vi "Game of Life.vi"() -> ()   [LabVIEW 2021, in "Game of Life.lvlib"]
doc: "InstrumentStudio plug-in example that displays Conway's Game of Life simulation in a graph."
uses:
  Game of Life.lvlib
  <vilib>/Plug-In SDKs/InstrumentStudio/Plugin Events Enum.ctl
  Helpers/Data Cluster.ctl
  Helpers/Configuration.ctl
  Queue Driver/Queue Operations.ctl
  Queue Driver/Queue State and Data.ctl
  User Event Driver/User Event Operations.ctl
  Helpers/Graph Elements.ctl
  <vilib>/Utility/error.llb/DialogType.ctl
  <vilib>/Utility/error.llb/Error Cluster From Error Code.vi
  <vilib>/ErrorRing/Error Ring.xnode
  <vilib>/Plug-In SDKs/InstrumentStudio/Plugin Session.lvclass
  <vilib>/Plug-In SDKs/InstrumentStudio/InstrumentStudio Plugin SDK.lvlib
  Queue Driver/Queue Driver.lvlib
  User Event Driver/User Event Driver.lvlib
panel:
  in  "Tab Control":enum32{"Game Panel", "Events"}(tab)
  in  "width":u32=100 caption="Board width" min=5 max=1000 step=1
  in  "height":u32=100 caption="Board height" min=5 max=1000 step=1
  in  "update interval":u32=500 caption="Update interval (msec)" min=100 max=2000 step=100
  out "generation":u32 caption="Generation"
  out "game of life":T1(graph)
  in  "Start/Stop":bool
  out "Event Record":i32(listbox)=-1
  in  "Session Id":u64
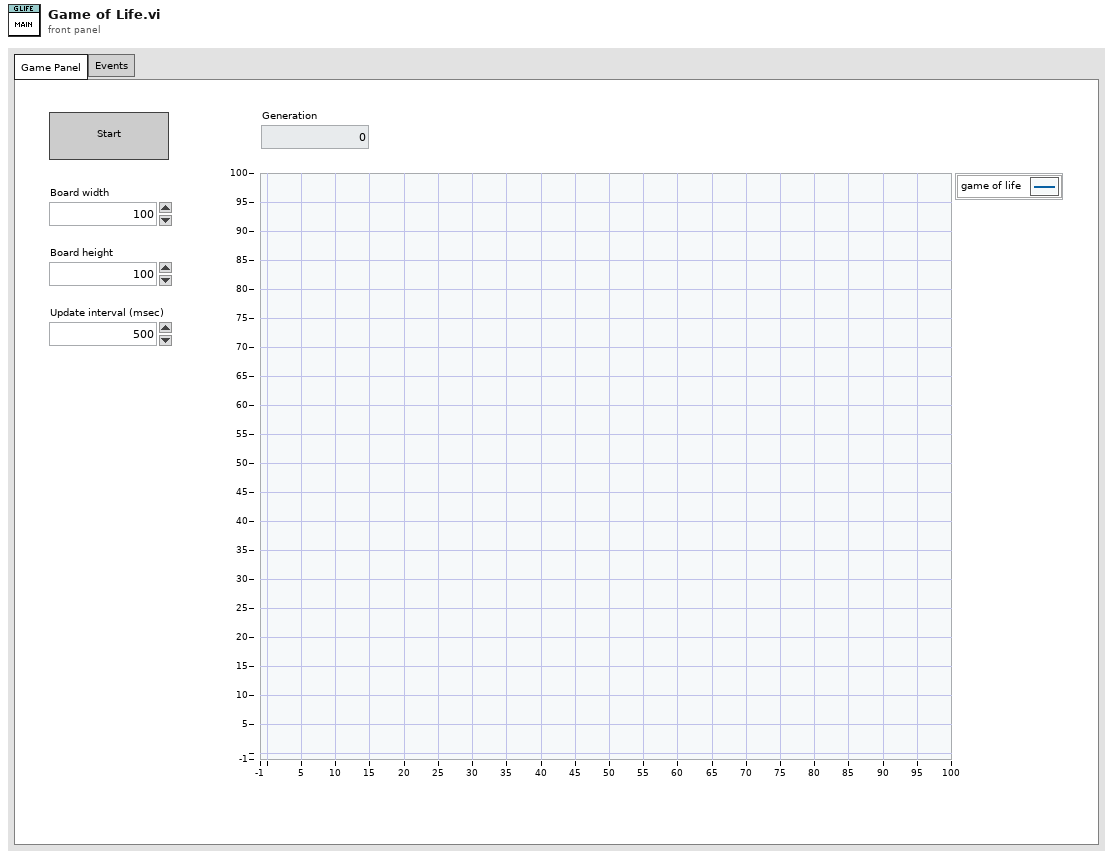
[diagram p1: front panel]
types:
  T1 = typedef "Game of Life.lvlib/Graph Elements.ctl" = cluster{"x data":dbl[], "y data":dbl[]}
  T2 = typedef "Game of Life.lvlib/User Event Driver.lvlib/User Event Operations.ctl" = enum16{"Create", "Destroy", "Get Reference", "Generate"}
  T3 = typedef "Game of Life.lvlib/Queue Driver.lvlib/Queue State and Data.ctl" = cluster{"state":string, "data":variant}
  T4 = typedef "Game of Life.lvlib/Queue Driver.lvlib/Queue Operations.ctl" = enum16{"Create Q", "Enqueue", "Enqueue N", "Enstack", "Enstack N", "Dequeue", "Flush", "Release"}
  T5 = typedef "Game of Life.lvlib/Data Cluster.ctl" = cluster{"configuration":T6, "generation":u32, "cells":bool[][], "event records":string[], "running?":bool, "board update time":timestamp}
  T6 = typedef "Game of Life.lvlib/Configuration.ctl" = cluster{"height":u32, "width":u32, "interval":u32}
  T7 = typedef "InstrumentStudio Plugin SDK.lvlib/Plugin Events Enum.ctl" = enum32{"Shutdown", "Project Saved", "Stop All Outputs", "Generic Message", "Active Pin Map Changed", "Selected Sites Changed"}
  T8 = typedef "InstrumentStudio Plugin SDK.lvlib/Event Registration Refnum.ctl" = refnum<event-registration>
  T9 = cluster{"Event Refnum":T8, "Event Registration Refnum":refnum<event-registration>}
  T10 = enum8{"Enabled", "Disabled", "Disabled and Grayed Out"}
  T11 = typedef "DialogType.ctl" = u16
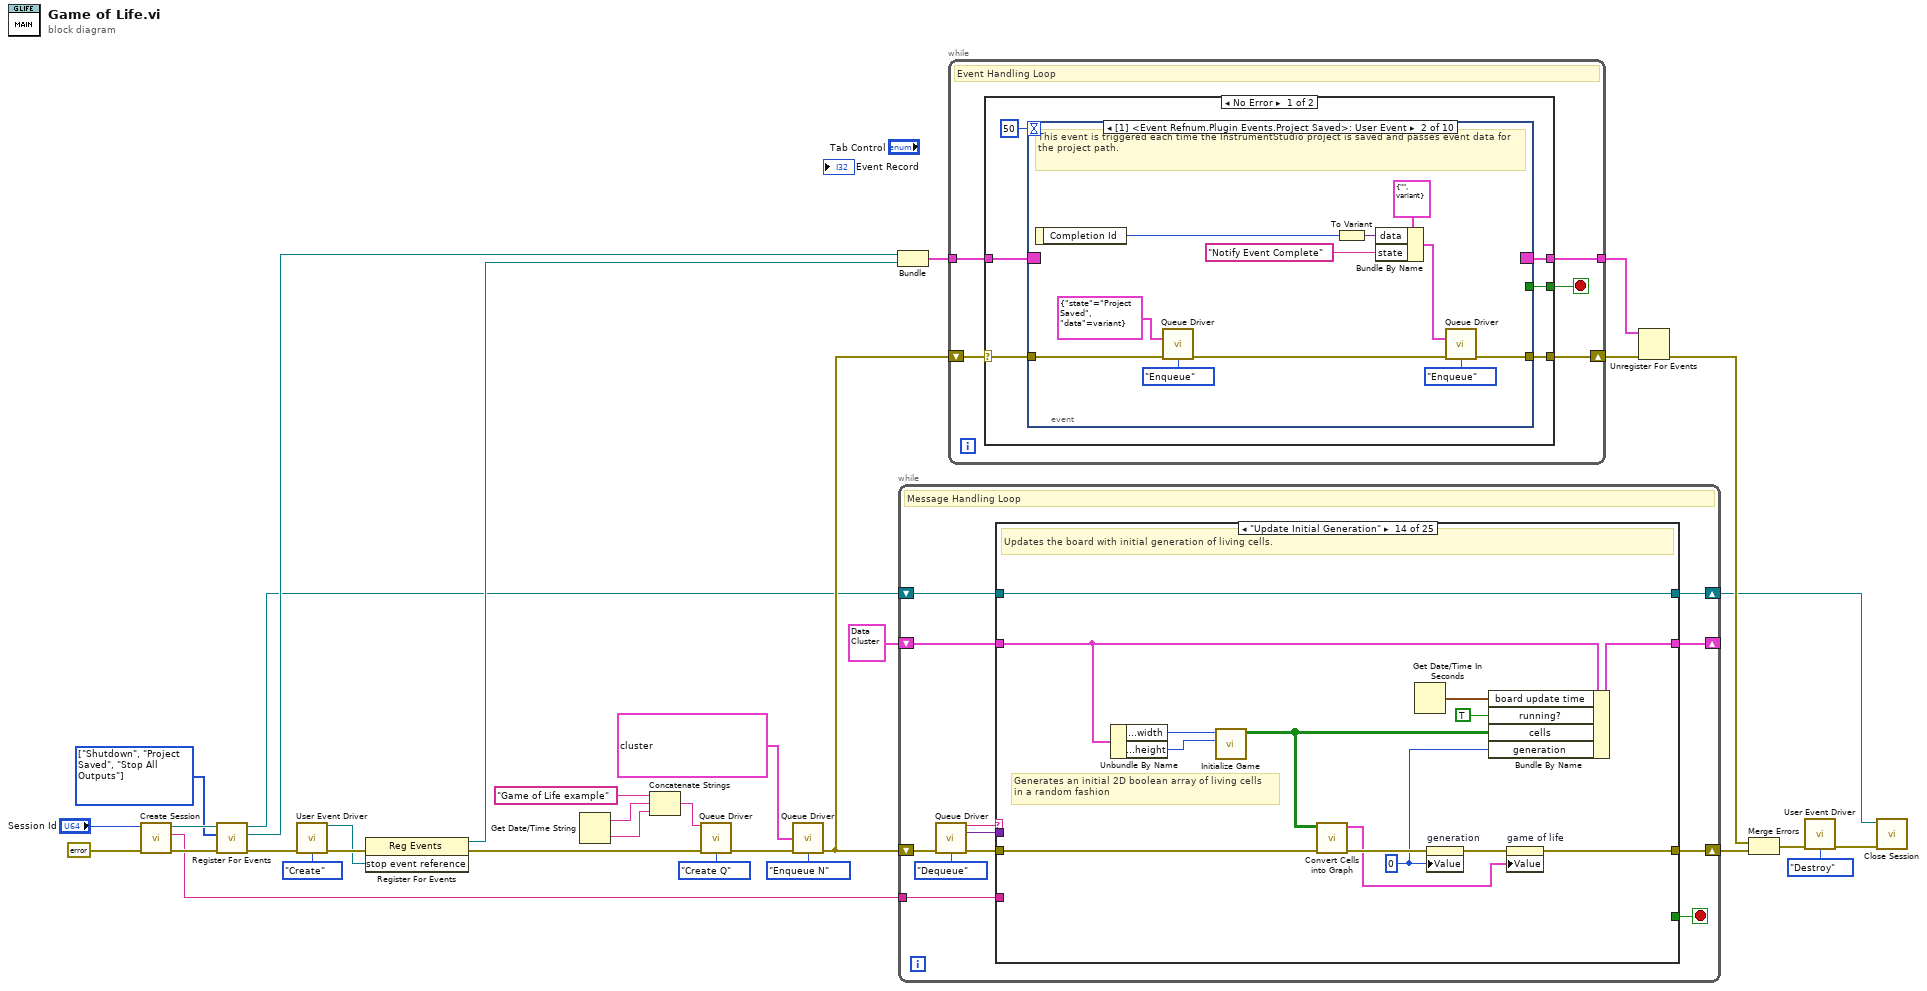
[diagram p0: block diagram]
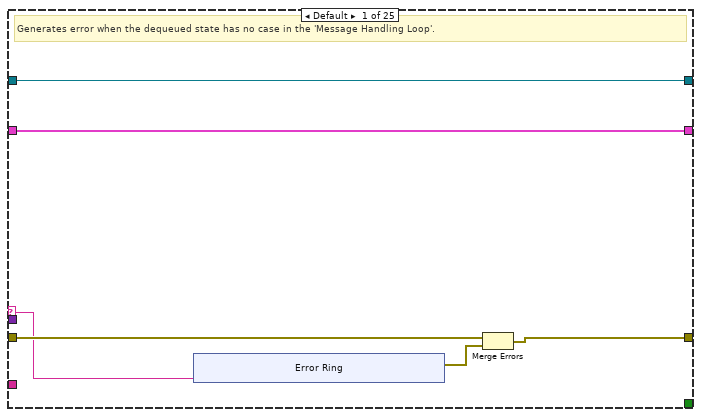
[diagram p2: hidden frame]
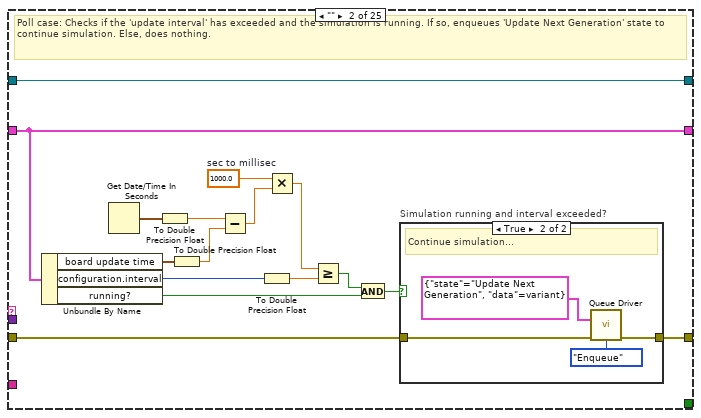
[diagram p3: hidden frame]
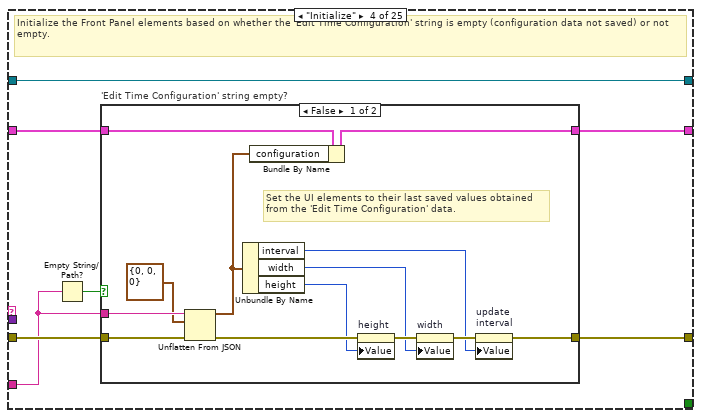
[diagram p6: hidden frame]
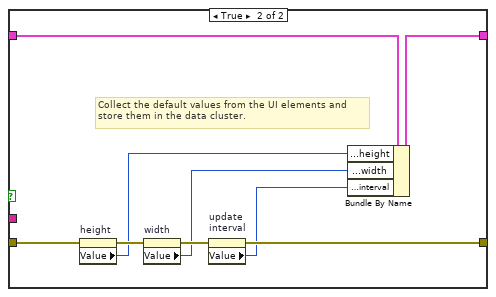
[diagram p7: hidden frame]
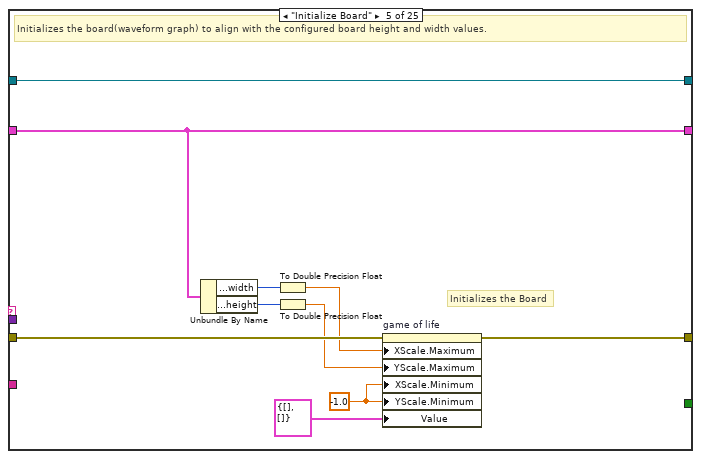
[diagram p8: hidden frame]
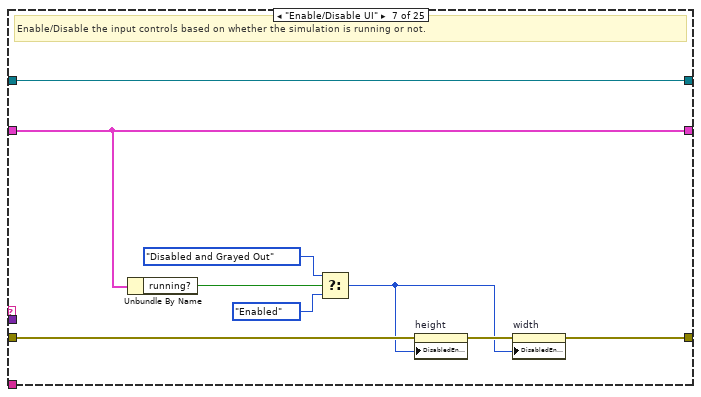
[diagram p10: hidden frame]
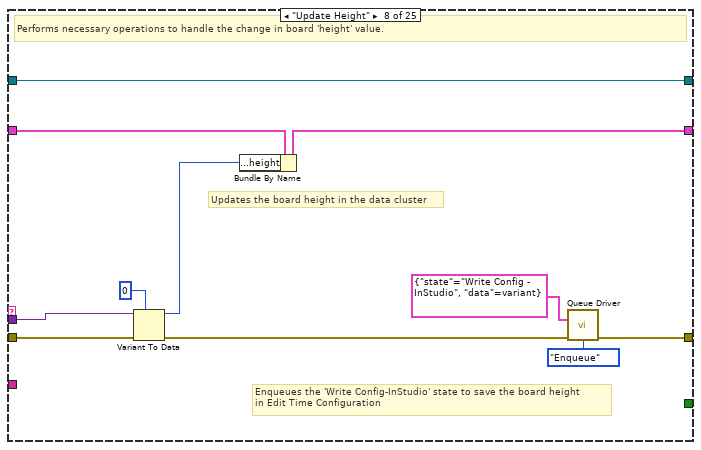
[diagram p11: hidden frame]
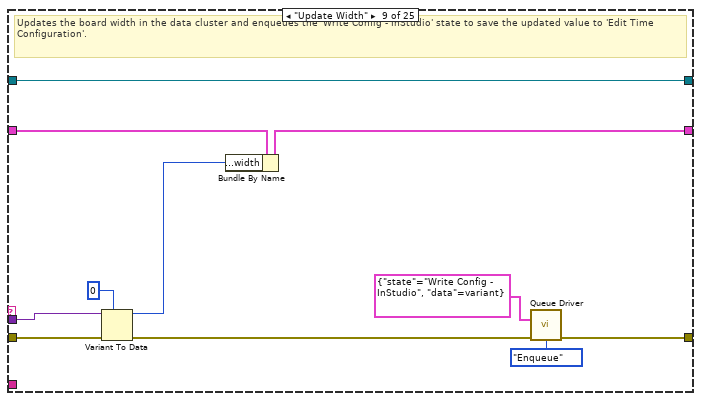
[diagram p12: hidden frame]
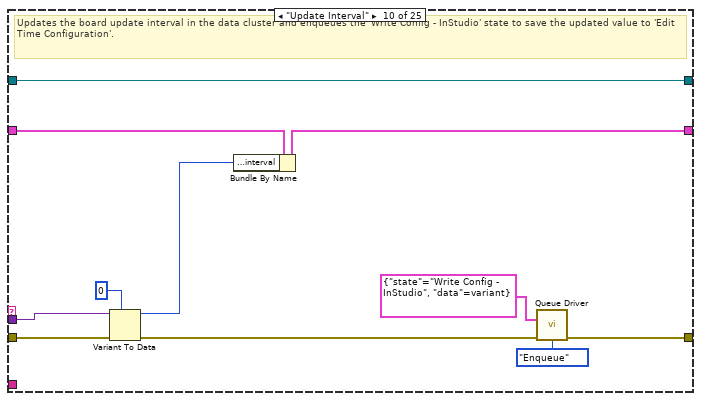
[diagram p13: hidden frame]
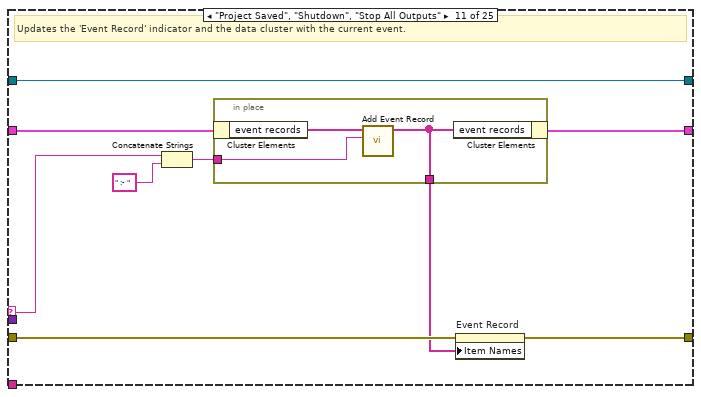
[diagram p14: hidden frame]
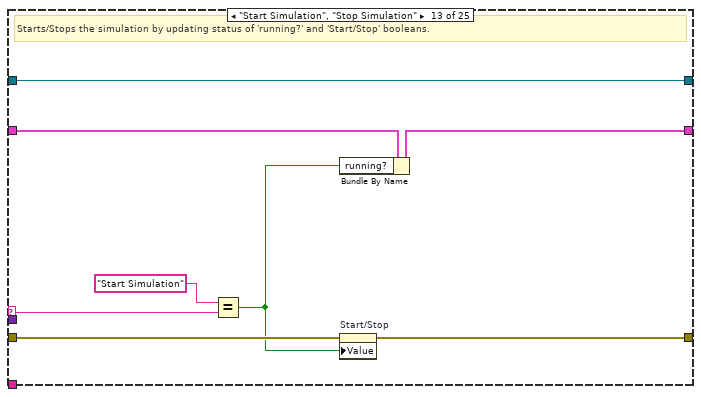
[diagram p16: hidden frame]
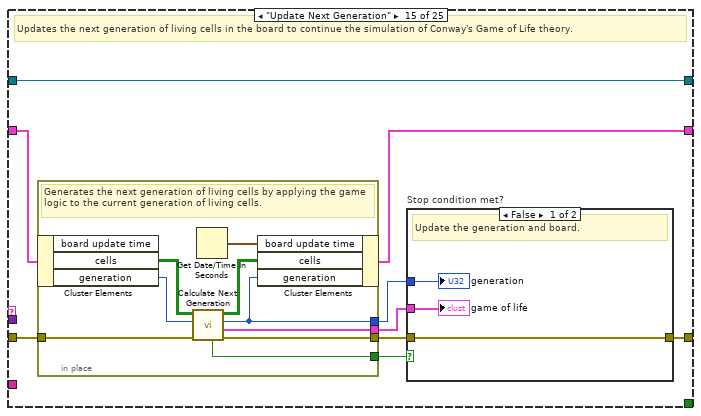
[diagram p17: hidden frame]
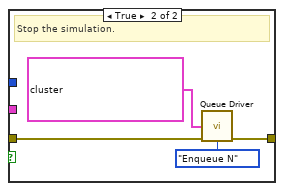
[diagram p18: hidden frame]
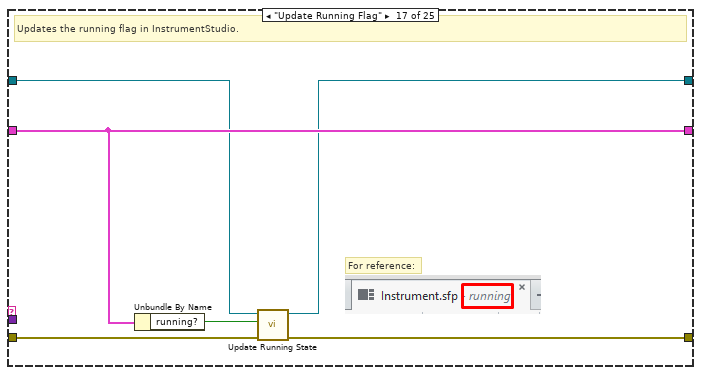
[diagram p20: hidden frame]
diagram:
  w24 = T7[] [enum."Shutdown", enum."Project Saved", enum."Stop All Outputs"] items=["Shutdown", "Project Saved", "Stop All Outputs", "Generic Message", "Active Pin Map Changed", "Selected Sites Changed"] ("Events To Register")
  n1 = call <vilib>:"Create Session.vi"("error in (no error)"=errorcluster {"status"=FALSE, "code"=0, "source"=""}, "Session Id"="Session Id") -> ("error out"=w13:errorcluster, "Edit Time Configuration"=w5:string, "Session out"=w25:refnum<class "Plugin Session.lvclass">)  [unwired: 5 in, 2 out]
  n2 = call <vilib>:"Register For Events.vi"("error in (no error)"=w13, "Events To Register"=w24, "Session in"=w25) -> ("error out"=w12:errorcluster, "Event Refnum"=w23:T8, "Session out"=w7:refnum<class "Plugin Session.lvclass">)  [unwired: 6 in]
  n3 = call "User Event Driver.vi"("error in"=w12, "user event operation"=User_Event_Operations."Create" ("LV2 Operation")) -> ("stop event reference"=w10:refnum<user-event>, "error out"=w11:errorcluster)  [unwired: 12 in]
  n4 = register-events(error in=w11, w10) -> (reference out=w22:refnum<event-registration>, error out=w21:errorcluster)  [unwired: 1 in]
  n5 = Get Date/Time String() -> (date string=w31:string, time string=w32:string)  [unwired: 3 in]
  n6 = Concatenate Strings("Game of Life example" ("Name"), w31, w32) -> (w27:string)
  n7 = call "Queue Driver.vi"("queue name"=w27, "error in"=w21, "queue operation"=Queue_Operations."Create Q" ("Queue Operations")) -> ("error out"=w28:errorcluster)  [unwired: 10 in, 2 out]
  n8 = call "Queue Driver.vi"("array of state and data"=T3[] [{"state"="Initialize", "data"=variant}, {"state"="Initialize Board", "data"=variant}, {"state"="Enable/Disable UI", "data"=variant}] ("Array of State and Data"), "error in"=w28, "queue operation"=Queue_Operations."Enqueue N" ("Queue Operations")) -> ("error out"=w8:errorcluster)  [unwired: 10 in, 2 out]
  n9 = Bundle("Event Refnum"=w23, "Event Registration Refnum"=w22) -> (w1:T9)  [unwired: 1 in]
  n10 = while {
    shift-right: [w37] -> w17
    shift-left: w8 -> [w45]
    shift-right: [w42] -> _
    shift-left: T5 {"configuration"={"height"=0, "width"=0, "interval"=0}, "generation"=0, "cells"=[], "event records"=[], "running?"=FALSE, "board update time"=timestamp(0 s since 1904-01-01)} ("Data") -> [w38]
    shift-right: [w41] -> w18
    shift-left: w7 -> [w40]
    tunnel: w5 -> [w35]
    stop <- w39 stop-if-true
    # "Message Handling Loop"
    n11 = call "Queue Driver.vi"("error in"=w45, "queue operation"=Queue_Operations."Dequeue" ("Queue Operations")) -> ("dequeued state"=w34:string, "dequeued data"=w36:variant, "error out"=w44:errorcluster)  [unwired: 11 in]
    n12 = case shown="\"Update Initial Generation\"" w34 {
      selector: w34 -> [w46 _ _ _ _ _ _ _ _ _ w170 _ w183 _ _ _ _ _ _ _ _ _ _ _ _]
      tunnel: w40 -> [w47 w74 w80 w85 w121 w122 w133 w144 w155 w166 w167 w179 w189 w203 w212 w229 w233 w241 w252 w256 w271 w289 w293 w302 w318]
      tunnel: [w49 w73 w82 w84 w118 w124 w125 w135 w145 w156 w174 w181 w187 w200 w209 w231 w236 w244 w253 w258 w265 w285 w295 w297 w311] -> w37
      tunnel: w44 -> [w51 w72 w82 w89 w120 w124 w132 w143 w154 w165 w175 w181 w188 w199 w211 w231 w237 w246 w255 w258 w262 w281 w295 w298 w317]
      tunnel: w38 -> [w48 w63 w81 w88 w113 w123 w130 w140 w151 w162 w169 w180 w185 w196 w210 w230 w235 w242 w254 w257 w260 w276 w294 w303 w319]
      tunnel: [w48 w63 w81 w87 w113 w123 w130 w139 w150 w161 w168 w180 w186 w201 w208 w230 w235 w242 w254 w257 w259 w275 w294 w303 w319] -> w42
      tunnel: [w47 w74 w80 w85 w121 w122 w133 w144 w155 w166 w167 w179 w189 w203 w212 w229 w232 w240 w251 w256 w271 w289 w293 w302 w318] -> w41
      tunnel: [_ _ _ _ _ _ _ _ _ _ _ _ _ _ _ _ _ _ _ _ _ _ _ _ TRUE] -> w39
      tunnel: w36 -> [_ _ _ _ _ _ _ w141 w152 w163 _ _ _ _ _ _ _ _ w249 _ _ w284 _ _ _]
      tunnel: w35 -> [_ _ _ w83 _ _ _ _ _ _ _ _ _ _ _ _ _ _ _ _ _ _ _ _ _]
      frame Default {
        # "Generates error when the dequeued state has no case in the 'Message Handling Loop'."
        n13 = xnode "Error Ring"("parameter 0"=w46) -> ("error out"=w50:errorcluster)
        n14 = Merge Errors(w51, w50) -> (w49:errorcluster)
      }
      frame "" {
        w69 = 1000.0  # sec to millisec
        # "Poll case: Checks if the 'update interval' has exceeded and the simulation is running. If so, enqueues 'Update Next Generation' state to continue simulation. Else, does nothing."
        n15 = Unbundle By Name(w63) -> ("board update time"=w65:timestamp, "configuration.interval"=w60:u32, "running?"=w62:bool)
        n16 = Get Date/Time In Seconds() -> (seconds since 1Jan1904=w64:timestamp)
        n17 = To Double Precision Float(number=w64) -> (double precision float=w70:dbl)
        n18 = To Double Precision Float(number=w65) -> (double precision float=w71:dbl)
        n19 = Subtract(x=w70, y=w71) -> (x-y=w68:dbl)
        n20 = To Double Precision Float(number=w60) -> (double precision float=w66:dbl)
        n21 = Multiply(x=w69, y=w68) -> (x*y=w67:dbl)
        n22 = Greater Or Equal?(x=w67, y=w66) -> (x >= y?=w61:bool)
        n23 = And(x=w61, y=w62) -> (x .and. y?=w59:bool)
        n24 = case "Simulation running and interval exceeded?" shown="True" w59 {
          tunnel: w72 -> [w75 w78]
          tunnel: [w75 w77] -> w73
          frame False {
            # "Pass"
          }
          frame True {
            # "Continue simulation..."
            n25 = call "Queue Driver.vi"("state and data"=T3 {"state"="Update Next Generation", "data"=variant} ("State and Data"), "error in"=w78, "queue operation"=Queue_Operations."Enqueue" ("Queue Operations")) -> ("error out"=w77:errorcluster)  [unwired: 10 in, 2 out]
          }
        }
      }
      frame "*****Initialization*****" {
      }
      frame "Initialize" {
        # "Initialize the Front Panel elements based on whether the 'Edit Time Configuration' string is empty (configuration data not saved) or not empty."
        n26 = Empty String/Path?(string/path=w83) -> (empty?=w86:bool)
        n27 = case "'Edit Time Configuration' string empty?" shown="False" w86 {
          tunnel: w89 -> [w96 w111]
          tunnel: w88 -> [w98 w108]
          tunnel: [w97 w107] -> w87
          tunnel: [w92 w104] -> w84
          tunnel: w83 -> [w91 _]
          frame False {
            # "Set the UI elements to their last saved values obtained\nfrom the 'Edit Time Configuration' data."
            n28 = Unflatten From JSON(JSON string=w91, type and defaults=T6 {"height"=0, "width"=0, "interval"=0} ("Configuration"), error in (no error)=w96) -> (value=w94:T6, error out=w95:errorcluster)  [unwired: 4 in]
            n29 = Unbundle By Name(w94) -> ("interval"=w100:u32, "width"=w99:u32, "height"=w93:u32)
            n30 = Bundle By Name(cluster=w98, "configuration"=w94) -> (w97:T5)
            n31 = property on="height" class="DigNum (strict)"(error in=w95, "Value"=w93) -> (error out=w101:errorcluster)  [unwired: 1 in, 1 out]
            n32 = property on="width" class="DigNum (strict)"(error in=w101, "Value"=w99) -> (error out=w102:errorcluster)  [unwired: 1 in, 1 out]
            n33 = property on="update\ninterval" class="DigNum (strict)"(error in=w102, "Value"=w100) -> (error out=w92:errorcluster)  [unwired: 1 in, 1 out]
          }
          frame True {
            # "Collect the default values from the UI elements and\nstore them in the data cluster."
            n34 = property on="height" class="DigNum (strict)"(error in=w111) -> (error out=w109:errorcluster, "Value"=w106:u32)  [unwired: 1 in, 1 out]
            n35 = property on="width" class="DigNum (strict)"(error in=w109) -> (error out=w110:errorcluster, "Value"=w105:u32)  [unwired: 1 in, 1 out]
            n36 = property on="update\ninterval" class="DigNum (strict)"(error in=w110) -> (error out=w104:errorcluster, "Value"=w103:u32)  [unwired: 1 in, 1 out]
            n37 = Bundle By Name(cluster=w108, "configuration.height"=w106, "configuration.width"=w105, "configuration.interval"=w103) -> (w107:T5)
          }
        }
      }
      frame "Initialize Board" {
        w119 = -1.0 ("Y Scale.Range:Minimum")
        # "Initializes the Board"
        # "Initializes the board(waveform graph) to align with the configured board height and width values."
        n38 = Unbundle By Name(w113) -> ("configuration.width"=w117:u32, "configuration.height"=w116:u32)
        n39 = To Double Precision Float(number=w117) -> (double precision float=w115:dbl)
        n40 = To Double Precision Float(number=w116) -> (double precision float=w114:dbl)
        n41 = property on="game of life" class="XYGraph (strict)"(error in=w120, "XScale.Maximum"=w115, "YScale.Maximum"=w114, "XScale.Minimum"=w119, "YScale.Minimum"=w119, "Value"=T1 {"x data"=[], "y data"=[]} ("game of life")) -> (error out=w118:errorcluster)  [unwired: 1 in, 1 out]
      }
      frame "*****Front Panel Updates*****" {
      }
      frame "Enable/Disable UI" {
        # "Enable/Disable the input controls based on whether the simulation is running or not."
        n42 = Unbundle By Name(w130) -> ("running?"=w129:bool)
        n43 = Select(t=T10."Disabled and Grayed Out", s=w129, f=T10."Enabled" ("Disabled")) -> (s? t:f=w126:T10)
        n44 = property on="height" class="DigNum (strict)"(error in=w132, "DisabledEnum"=w126) -> (error out=w131:errorcluster)  [unwired: 1 in, 1 out]
        n45 = property on="width" class="DigNum (strict)"(error in=w131, "DisabledEnum"=w126) -> (error out=w125:errorcluster)  [unwired: 1 in, 1 out]
      }
      frame "Update Height" {
        # "Enqueues the 'Write Config-InStudio' state to save the board height\nin Edit Time Configuration"
        # "Updates the board height in the data cluster"
        # "Performs necessary operations to handle the change in board 'height' value."
        n46 = Variant To Data(error in=w143, type=u32 0, Variant=w141) -> (data=w138:u32, error out=w134:errorcluster)
        n47 = Bundle By Name(cluster=w140, "configuration.height"=w138) -> (w139:T5)
        n48 = call "Queue Driver.vi"("state and data"=T3 {"state"="Write Config - InStudio", "data"=variant} ("State and Data"), "error in"=w134, "queue operation"=Queue_Operations."Enqueue" ("Queue Operations")) -> ("error out"=w135:errorcluster)  [unwired: 10 in, 2 out]
      }
      frame "Update Width" {
        # "Updates the board width in the data cluster and enqueues the 'Write Config - InStudio' state to save the updated value to 'Edit Time Configuration'."
        n49 = Variant To Data(error in=w154, type=u32 0, Variant=w152) -> (data=w149:u32, error out=w146:errorcluster)
        n50 = Bundle By Name(cluster=w151, "configuration.width"=w149) -> (w150:T5)
        n51 = call "Queue Driver.vi"("state and data"=T3 {"state"="Write Config - InStudio", "data"=variant} ("State and Data"), "error in"=w146, "queue operation"=Queue_Operations."Enqueue" ("Queue Operations")) -> ("error out"=w145:errorcluster)  [unwired: 10 in, 2 out]
      }
      frame "Update Interval" {
        # "Updates the board update interval in the data cluster and enqueues the 'Write Config - InStudio' state to save the updated value to 'Edit Time Configuration'."
        n52 = Variant To Data(error in=w165, type=u32 0, Variant=w163) -> (data=w160:u32, error out=w157:errorcluster)
        n53 = Bundle By Name(cluster=w162, "configuration.interval"=w160) -> (w161:T5)
        n54 = call "Queue Driver.vi"("state and data"=T3 {"state"="Write Config - InStudio", "data"=variant} ("State and Data"), "error in"=w157, "queue operation"=Queue_Operations."Enqueue" ("Queue Operations")) -> ("error out"=w156:errorcluster)  [unwired: 10 in, 2 out]
      }
      frame "Project Saved", "Shutdown", "Stop All Outputs" {
        # "Updates the 'Event Record' indicator and the data cluster with the current event."
        n55 = Concatenate Strings(w170, " :- " ("string")) -> (w173:string)
        n56 = in-place {
          in-place-border: w173 -> [w178]
          in-place-border: [w176] -> w172
          n57 = in-place-cluster #1(w169) -> ("event records"=w177:string[])
          n58 = call "Add Event Record.vi"("event tag"=w178, "event records in"=w177) -> ("event records out"=w176:string[])  [unwired: 9 in]
          n59 = in-place-cluster #1("event records"=w176) -> (w168:T5)
        }
        n60 = property on="Event Record" class="LstBox (strict)"(error in=w175, "Item Names"=w172) -> (error out=w174:errorcluster)  [unwired: 1 in, 1 out]
      }
      frame "*****Implementation Logic*****" {
      }
      frame "Start Simulation", "Stop Simulation" {
        # "Starts/Stops the simulation by updating status of 'running?' and 'Start/Stop' booleans."
        n61 = Equal?(x="Start Simulation" ("y"), y=w183) -> (x = y?=w182:bool)
        n62 = Bundle By Name(cluster=w185, "running?"=w182) -> (w186:T5)
        n63 = property on="Start/Stop" class="Bool (strict)"(error in=w188, "Value"=w182) -> (error out=w187:errorcluster)  [unwired: 1 in, 1 out]
      }
      frame "Update Initial Generation" {
        w191 = u32 0 ("Generation")
        # "Generates an initial 2D boolean array of living cells\nin a random fashion"
        # "Updates the board with initial generation of living cells."
        n64 = Unbundle By Name(w196) -> ("configuration.width"=w202:u32, "configuration.height"=w195:u32)
        n65 = call "Initialize Game.vi"("height"=w195, "width"=w202) -> ("living cells"=w190:bool[][])  [unwired: 9 in]
        n66 = call "Convert Cells into Graph.vi"("error in"=w199, "cells in"=w190) -> ("error out"=w198:errorcluster, "graph elements"=w192:T1)  [unwired: 8 in]
        n67 = Get Date/Time In Seconds() -> (seconds since 1Jan1904=w194:timestamp)
        n68 = property on="generation" class="DigNum (strict)"(error in=w198, "Value"=w191) -> (error out=w197:errorcluster)  [unwired: 1 in, 1 out]
        n69 = Bundle By Name(cluster=w196, "board update time"=w194, "running?"=TRUE, "cells"=w190, "generation"=w191) -> (w201:T5)
        n70 = property on="game of life" class="XYGraph (strict)"(error in=w197, "Value"=w192) -> (error out=w200:errorcluster)  [unwired: 1 in, 1 out]
      }
      frame "Update Next Generation" {
        # "Updates the next generation of living cells in the board to continue the simulation of Conway's Game of Life theory."
        n71 = in-place {
          in-place-border: w211 -> [w228]
          in-place-border: [w227] -> w207
          in-place-border: [w222] -> w206
          in-place-border: [w223] -> w205
          in-place-border: [w220] -> w204
          # "Generates the next generation of living cells by applying the game logic to the current generation of living cells."
          n72 = in-place-cluster #2(w210) -> ("cells"=w224:bool[][], "generation"=w226:u32)  [unwired: 1 out]
          n73 = call "Calculate Next Generation.vi"("error in"=w228, "generation in"=w226, "cells in"=w224) -> ("error out"=w227:errorcluster, "graph elements"=w223:T1, "generation out"=w222:u32, "cells out"=w225:bool[][], "stop generation?"=w220:bool)  [unwired: 4 in]
          n74 = Get Date/Time In Seconds() -> (seconds since 1Jan1904=w221:timestamp)
          n75 = in-place-cluster #2("board update time"=w221, "cells"=w225, "generation"=w222) -> (w208:T5)
        }
        n76 = case "Stop condition met?" shown="False" w204 {
          tunnel: w207 -> [w215 w218]
          tunnel: [w215 w217] -> w209
          tunnel: w206 -> [w214 _]
          tunnel: w205 -> [w213 _]
          frame False {
            # "Update the generation and board."
            "generation" <- w214
            "game of life" <- w213
          }
          frame True {
            # "Stop the simulation."
            n77 = call "Queue Driver.vi"("array of state and data"=T3[] [{"state"="Stop Simulation", "data"=variant}, {"state"="Enable/Disable UI", "data"=variant}, {"state"="Update Running Flag", "data"=variant}] ("Array of State and Data"), "error in"=w218, "queue operation"=Queue_Operations."Enqueue N" ("Queue Operations")) -> ("error out"=w217:errorcluster)  [unwired: 10 in, 2 out]
          }
        }
      }
      frame "*****InstrumentStudio Interaction*****" {
      }
      frame "Update Running Flag" {
        # "For reference:"
        # "Updates the running flag in InstrumentStudio."
        n78 = Unbundle By Name(w235) -> ("running?"=w234:bool)
        n79 = call <vilib>:"Update Running State.vi"("error in (no error)"=w237, "Is Running"=w234, "Plugin Session in"=w233) -> ("error out"=w236:errorcluster, "Plugin Session out"=w232:refnum<class "Plugin Session.lvclass">)  [unwired: 7 in]
      }
      frame "Write Config - InStudio" {
        # "Saves the configuration values from the data cluster into the 'Edit Time Configuration' value of the current InstrumentStudio session."
        n80 = Unbundle By Name(w242) -> ("configuration"=w239:T6)
        n81 = Flatten To JSON(enable LabVIEW extensions? (T)=FALSE, anything=w239, error in (no error)=w246) -> (JSON string=w243:string, 11:w245:errorcluster)
        n82 = call <vilib>:"Write Edit Time Configuration.vi"("error in (no error)"=w245, "Edit Time Configuration"=w243, "Session in"=w241) -> ("error out"=w244:errorcluster, "Session out"=w240:refnum<class "Plugin Session.lvclass">)  [unwired: 7 in]
      }
      frame "Notify Event Complete" {
        # "Send acknowledgement to InstrumentStudio to notify the completion of event handling for the registered event using the 'Completion Id' (except for the 'Shutdown' event)."
        n83 = Variant To Data(error in=w255, type=i64 0, Variant=w249) -> (data=w247:i64, error out=w250:errorcluster)
        n84 = call <vilib>:"Notify Event Complete.vi"("error in (no error)"=w250, "Completion Id"=w247, "Session in"=w252) -> ("error out"=w253:errorcluster, "Session out"=w251:refnum<class "Plugin Session.lvclass">)  [unwired: 7 in]
      }
      frame "*****Error Handling*****" {
      }
      frame "Error" {
        w270 = T11 0 items=["no dialog", "OK message", "continue or stop message", "OK message + warnings", "continue/stop + warnings"] ("type of dialog (OK msg:1)")
        # "Log error in the 'Event Record'"
        # "Performs the necessary error handling for any error encountered in 'Message Handling Loop'."
        n85 = call <vilib>:"Simple Error Handler.vi"("type of dialog (OK msg:1)"=w270, "error in (no error)"=w262) -> ("error out"=w266:errorcluster, "message"=w264:string)  [unwired: 3 in, 3 out]
        n86 = call "Align Error Message.vi"("message in"=w264) -> ("message out"=w269:string)  [unwired: 10 in]
        n87 = Concatenate Strings(w269, " :- " ("string")) -> (w267:string)
        n88 = in-place {
          in-place-border: w267 -> [w273]
          in-place-border: [w272] -> w261
          n89 = in-place-cluster #3(w260) -> ("event records"=w274:string[])
          n90 = call "Add Event Record.vi"("event tag"=w273, "event records in"=w274) -> ("event records out"=w272:string[])  [unwired: 9 in]
          n91 = in-place-cluster #3("event records"=w272) -> (w259:T5)
        }
        n92 = call <vilib>:"Clear Errors.vi"("error in (no error)"=w266) -> ("error out"=w263:errorcluster)  [unwired: 5 in, 1 out]
        n93 = property on="Event Record" class="LstBox (strict)"(error in=w263, "Item Names"=w261) -> (error out=w265:errorcluster)  [unwired: 1 in, 1 out]
      }
      frame "Event Handler Error" {
        w283 = T11 0 items=["no dialog", "OK message", "continue or stop message", "OK message + warnings", "continue/stop + warnings"] ("type of dialog (OK msg:1)")
        # "Log error in the 'Event Record'"
        # "Performs the necessary error handling for any error encountered in 'Event Handling Loop'."
        n94 = Variant To Data(error in=w281, type=errorcluster {"status"=FALSE, "code"=0, "source"=""} ("error out"), Variant=w284) -> (data=w278:errorcluster, error out=w280:errorcluster)
        n95 = call <vilib>:"Simple Error Handler.vi"("type of dialog (OK msg:1)"=w283, "error in (no error)"=w278) -> ("message"=w282:string)  [unwired: 3 in, 4 out]
        n96 = call "Align Error Message.vi"("message in"=w282) -> ("message out"=w288:string)  [unwired: 10 in]
        n97 = Concatenate Strings(w288, " :- " ("string")) -> (w286:string)
        n98 = in-place {
          in-place-border: w286 -> [w291]
          in-place-border: [w290] -> w277
          n99 = in-place-cluster #4(w276) -> ("event records"=w292:string[])
          n100 = call "Add Event Record.vi"("event tag"=w291, "event records in"=w292) -> ("event records out"=w290:string[])  [unwired: 9 in]
          n101 = in-place-cluster #4("event records"=w290) -> (w275:T5)
        }
        n102 = property on="Event Record" class="LstBox (strict)"(error in=w280, "Item Names"=w277) -> (error out=w285:errorcluster)  [unwired: 1 in, 1 out]
      }
      frame "*****Exit Operations*****" {
      }
      frame "Confirm Quit" {
        # "Displays a pop-up to the user to confirm whether the user is sure about quitting."
        n103 = Two Button Dialog(message="Are you sure you want to quit?", 1:"No, continue" ("F button name (\"Cancel\")"), 2:"Yes, quit" ("T button name (\"OK\")")) -> (T button?=w296:bool)
        n104 = case "Quit execution?" shown="True" w296 {
          tunnel: w298 -> [w304 w306]
          tunnel: [w304 w305] -> w297
          frame False {
            # "Continue..."
          }
          frame True {
            # "Exit the application."
            n105 = call "Queue Driver.vi"("array of state and data"=T3[] [{"state"="Stop Simulation", "data"=variant}, {"state"="Enable/Disable UI", "data"=variant}, {"state"="Update Running Flag", "data"=variant}, {"state"="Exit", "data"=variant}] ("Array of State and Data"), "error in"=w306, "queue operation"=Queue_Operations."Enqueue N" ("Queue Operations")) -> ("error out"=w305:errorcluster)  [unwired: 10 in, 2 out]
          }
        }
      }
      frame "Exit" {
        # "Performs the necessary exit operations."
        n106 = property on="Event Record" class="LstBox (strict)"(error in=w317, "Item Names"=string[] []) -> (error out=w314:errorcluster)  [unwired: 1 in, 1 out]
        n107 = invoke class="VI" method="Default Vals.Reinit All"(error in=w314) -> (error out=w313:errorcluster)  [unwired: 2 in, 2 out]
        n108 = call "User Event Driver.vi"("error in"=w313, "user event operation"=User_Event_Operations."Generate" ("LV2 Operation")) -> ("error out"=w312:errorcluster)  [unwired: 12 in, 1 out]
        n109 = call "Queue Driver.vi"("error in"=w312, "queue operation"=Queue_Operations."Release" ("Queue Operations")) -> ("error out"=w311:errorcluster)  [unwired: 11 in, 2 out]
      }
    }
  }
  n110 = while {
    tunnel: w1 -> [w321]
    shift-right: [w323] -> w20
    shift-left: w8 -> [w324]
    tunnel: [w322] -> w9
    stop <- w320 stop-if-true
    # "Event Handling Loop"
    n111 = case shown="No Error" w324 {
      selector: w324 -> [w330 w402]
      tunnel: [w329 w407] -> w323
      tunnel: [w328 _] -> w322
      tunnel: w321 -> [w327 _]
      tunnel: [w326 _] -> w320
      frame No Error {
        n112 = event shown="[1] <Event Refnum.Plugin Events.Project Saved>: User Event" {
          selector: w327 -> [_ _ _ _ _ _ _ _ _ _]
          dyn-events: [_ _ _ _ _ _ _ _ _ _] -> w328
          timeout: 50 -> [_ _ _ _ _ _ _ _ _ _]
          tunnel: [w331 w337 w344 w357 w359 w367 w375 w383 w386 w397] -> w329
          tunnel: w330 -> [w331 w339 w346 w354 w359 w365 w373 w381 w385 w398]
          tunnel: [_ _ _ _ w358 _ _ _ _ _] -> w326
          event Timeout {
            n113 = event-data() -> ()  [unwired: 1 in, 1 out]
          }
          event User Event {
            # "This event is triggered each time the InstrumentStudio project is saved and passes event data for the project path."
            n114 = event-data() -> ("Completion Id"=w335:i64)  [unwired: 1 in]
            n115 = call "Queue Driver.vi"("state and data"=T3 {"state"="Project Saved", "data"=variant} ("State"), "error in"=w339, "queue operation"=Queue_Operations."Enqueue" ("Queue Operations")) -> ("error out"=w338:errorcluster)  [unwired: 10 in, 2 out]
            n116 = To Variant(anything=w335) -> (Variant=w334:variant)
            n117 = Bundle By Name(cluster=T3 {"state"="", "data"=variant} ("State and Data"), "data"=w334, "state"="Notify Event Complete" ("State")) -> (w340:T3)
            n118 = call "Queue Driver.vi"("state and data"=w340, "error in"=w338, "queue operation"=Queue_Operations."Enqueue" ("Queue Operations")) -> ("error out"=w337:errorcluster)  [unwired: 10 in, 2 out]
          }
          event User Event {
            # "The Stop All Outputs event is triggered when the 'Stop all outputs' button is pressed on the document toolbar."
            n119 = event-data() -> ("Completion Id"=w343:i64)  [unwired: 1 in]
            n120 = call "Queue Driver.vi"("array of state and data"=T3[] [{"state"="Stop All Outputs", "data"=variant}, {"state"="Stop Simulation", "data"=variant}, {"state"="Enable/Disable UI", "data"=variant}, {"state"="Update Running Flag", "data"=variant}] ("Array of State and Data"), "error in"=w346, "queue operation"=Queue_Operations."Enqueue N" ("Queue Operations")) -> ("error out"=w345:errorcluster)  [unwired: 10 in, 2 out]
            n121 = To Variant(anything=w343) -> (Variant=w348:variant)
            n122 = Bundle By Name(cluster=T3 {"state"="", "data"=variant} ("State and Data"), "data"=w348, "state"="Notify Event Complete" ("State")) -> (w350:T3)
            n123 = call "Queue Driver.vi"("state and data"=w350, "error in"=w345, "queue operation"=Queue_Operations."Enqueue" ("Queue Operations")) -> ("error out"=w344:errorcluster)  [unwired: 10 in, 2 out]
          }
          event User Event; Application Instance Close {
            # "This event doesn't need acknowledgment from plugin"
            # "The Shutdown event is triggered when the document containing the plugin is closed, the project containing the plugin is closed, or the plugin panel is removed from the document using the Edit Layout dialog."
            n124 = event-data() -> ()  [unwired: 1 in, 1 out]
            n125 = call "Queue Driver.vi"("array of state and data"=T3[] [{"state"="Shutdown", "data"=variant}, {"state"="Stop Simulation", "data"=variant}, {"state"="Enable/Disable UI", "data"=variant}, {"state"="Update Running Flag", "data"=variant}, {"state"="Exit", "data"=variant}] ("Array of State and Data"), "error in"=w354, "queue operation"=Queue_Operations."Enqueue N" ("Queue Operations")) -> ("error out"=w357:errorcluster)  [unwired: 10 in, 2 out]
          }
          event User Event {
            w358 = TRUE  # Stop execution
            # "The 'Message Handling Loop' encountered the \"Exit\" state which triggered this event to stop the 'Event Handling Loop'."
            n126 = event-data() -> ()  [unwired: 1 in, 1 out]
          }
          event "height": Value Change {
            # "Captures value change in 'height' and sends data to 'Message Handling Loop'."
            n127 = event-data() -> ("NewVal"=w363:u32)  [unwired: 1 in]
            n128 = To Variant(anything=w363) -> (Variant=w362:variant)
            n129 = Bundle By Name(cluster=T3 {"state"="", "data"=variant} ("State and Data"), "state"="Update Height" ("State"), "data"=w362) -> (w361:T3)
            n130 = call "Queue Driver.vi"("state and data"=w361, "error in"=w365, "queue operation"=Queue_Operations."Enqueue" ("Queue Operations")) -> ("error out"=w367:errorcluster)  [unwired: 10 in, 2 out]
          }
          event "width": Value Change {
            # "Captures value change in 'width' and sends data to 'Message Handling Loop'."
            n131 = event-data() -> ("NewVal"=w370:u32)  [unwired: 1 in]
            n132 = To Variant(anything=w370) -> (Variant=w369:variant)
            n133 = Bundle By Name(cluster=T3 {"state"="", "data"=variant} ("State and Data"), "state"="Update Width" ("State"), "data"=w369) -> (w368:T3)
            n134 = call "Queue Driver.vi"("state and data"=w368, "error in"=w373, "queue operation"=Queue_Operations."Enqueue" ("Queue Operations")) -> ("error out"=w375:errorcluster)  [unwired: 10 in, 2 out]
          }
          event "update interval": Value Change {
            # "Captures value change in 'update interval' and sends data to 'Message Handling Loop'."
            n135 = event-data() -> ("NewVal"=w378:u32)  [unwired: 1 in]
            n136 = To Variant(anything=w378) -> (Variant=w377:variant)
            n137 = Bundle By Name(cluster=T3 {"state"="", "data"=variant} ("State and Data"), "state"="Update Interval" ("State"), "data"=w377) -> (w376:T3)
            n138 = call "Queue Driver.vi"("state and data"=w376, "error in"=w381, "queue operation"=Queue_Operations."Enqueue" ("Queue Operations")) -> ("error out"=w383:errorcluster)  [unwired: 10 in, 2 out]
          }
          event "Start/Stop": Value Change {
            # "Captures value change in 'Start/Stop' button and enqueues the next state for the'Message Handling Loop' based on the new value of the button."
            n139 = event-data() -> ("NewVal"=w384:bool)  [unwired: 1 in]
            n140 = case shown="True" w384 {
              tunnel: [w388 w391] -> w386
              tunnel: w385 -> [w387 w392]
              frame True {
                n141 = call "Queue Driver.vi"("array of state and data"=T3[] [{"state"="Initialize Board", "data"=variant}, {"state"="Start Simulation", "data"=variant}, {"state"="Enable/Disable UI", "data"=variant}, {"state"="Update Running Flag", "data"=variant}, {"state"="Update Initial Generation", "data"=variant}] ("Array of State and Data"), "error in"=w387, "queue operation"=Queue_Operations."Enqueue N" ("Queue Operations")) -> ("error out"=w388:errorcluster)  [unwired: 10 in, 2 out]
              }
              frame False {
                n142 = call "Queue Driver.vi"("array of state and data"=T3[] [{"state"="Stop Simulation", "data"=variant}, {"state"="Enable/Disable UI", "data"=variant}, {"state"="Update Running Flag", "data"=variant}] ("Array of State and Data"), "error in"=w392, "queue operation"=Queue_Operations."Enqueue N" ("Queue Operations")) -> ("error out"=w391:errorcluster)  [unwired: 10 in, 2 out]
              }
            }
          }
          event Panel Close? {
            # "Send the 'Confirm Quit' message if the user closes the panel of the VI. Discard the event so the 'Confirm Quit' message has a chance to run."
            n143 = event-data() -> ()  [unwired: 1 in, 1 out]
            n144 = call "Queue Driver.vi"("state and data"=T3 {"state"="Confirm Quit", "data"=variant} ("State and Data"), "error in"=w398, "queue operation"=Queue_Operations."Enqueue" ("Queue Operations")) -> ("error out"=w397:errorcluster)  [unwired: 10 in, 2 out]
            n145 = event-data("Discard?"=TRUE) -> ()  [unwired: 1 in, 1 out]
          }
        }
      }
      frame Error {
        n146 = To Variant(anything=w402) -> (Variant=w401:variant)
        n147 = call <vilib>:"Clear Errors.vi"("error in (no error)"=w402) -> ("error out"=w400:errorcluster)  [unwired: 5 in, 1 out]
        n148 = Bundle By Name(cluster=T3 {"state"="", "data"=variant} ("state and data"), "state"="Event Handler Error", "data"=w401) -> (w404:T3)
        n149 = call "Queue Driver.vi"("state and data"=w404, "error in"=w400, "queue operation"=Queue_Operations."Enstack") -> ("error out"=w407:errorcluster)  [unwired: 10 in, 2 out]
      }
    }
  }
  n150 = Unregister For Events(event registration refnum=w9, error in=w20) -> (error out=w19:errorcluster)
  n151 = Merge Errors(w19, w17) -> (w4:errorcluster)
  n152 = call "User Event Driver.vi"("error in"=w4, "user event operation"=User_Event_Operations."Destroy" ("LV2 Operation")) -> ("error out"=w16:errorcluster)  [unwired: 12 in, 1 out]
  n153 = call <vilib>:"Close Session.vi"("error in (no error)"=w16, "Session in"=w18) -> ()  [unwired: 9 in, 1 out]
